vi "Test Day Total.vi"(8 "error in":errorcluster, 10 "Work Folder":path, 11 "Test Data Folder":path) -> (0 "error out":errorcluster, 2 "Report":string, 3 "Passed":bool)   [LabVIEW 2026]
doc: "Tests Day Total.vi and Day Total Entries.vi. Times are given as LOCAL date/time text and scanned here, so the daylight saving cases assume the US Central time zone of this computer (2026-11-01 has 25 hours, 2026-03-08 has 23).\n\nDay Total (entries built here): two finished entries add up; an entry crossing the next midnight counts only up to midnight; one started the previous evening counts only from midnight; a running entry counts up to Now and a later Now gives a larger total; overlapping entries are summed; 59.6 s rounds to 00:01:00 and 59 s stays 00:00:59; more than 24 h (overlaps) gives 25:00:00; on the 25-hour and the 23-hour day an entry from 00:00 to 23:59:59 and an entry spanning the whole day are clipped correctly; Now before the start counts 0; empty Entries gives 0 and 00:00:00.\n\nDay Total Entries (Test - Day Total Entries Cases.vi, on a copy of Test Data\\Samples with three entries added): an entry crossing local midnight is in the next day; the previous day is read from the previous month's file; a running entry from the previous day is included; the day's own entries come in start order; on the day after the 23-hour day 2026-03-08 (whose 24-hour read reaches into the next day) the entry is listed once; Day Total of each day's Total Entries; no error.\n\nInputs: Test Data Folder; Work Folder; error in. Outputs: Passed; Report; error out.\n\nGenerated by: Claude"
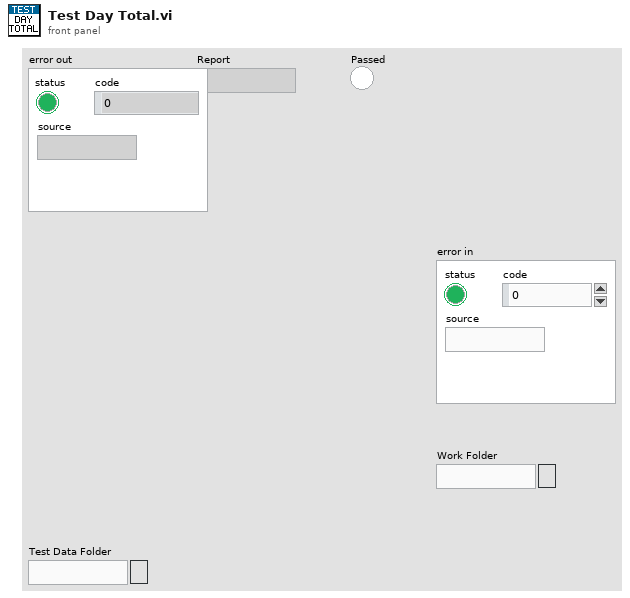
[diagram p1: front panel]
types:
  T1 = cluster{"ID":string, "Project ID":string, "Task ID":string, "Start Time":timestamp, "End Time":timestamp, "Description":string}
  T2 = cluster{"ID":string, "Project ID":string, "Task ID":string, "Start Time":timestamp, "End Time":timestamp, "Description":string}[]
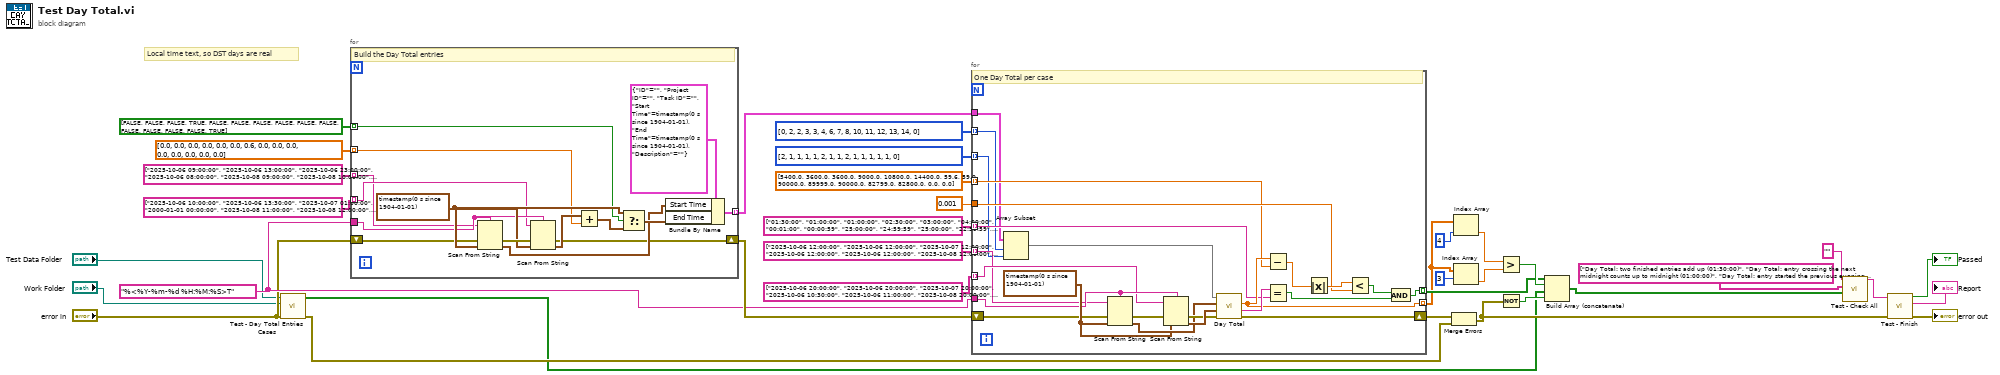
[diagram p0: block diagram]
diagram:
  w7 = "%<%Y-%m-%d %H:%M:%S>T" ("local time format")
  # "Local time text, so DST days are real"
  n1 = call "Test - Day Total Entries Cases.vi"("error in"="error in", "Work Folder"="Work Folder", "Test Data Folder"="Test Data Folder") -> ("error out"=w32:errorcluster, "Conditions"=w31:bool[])  [unwired: 7 in]
  n2 = for {
    tunnel: string[] ["2025-10-06 09:00:00", "2025-10-06 13:00:00", "2025-10-06 23:00:00", "2025-10-06 08:00:00", "2025-10-08 09:00:00", "2025-10-08 10:00:00", "2025-10-09 09:00:00", "2025-10-09 09:00:00", "2025-10-10 00:00:00", "2025-10-10 23:00:00", "2026-11-01 00:00:00", "2026-10-31 20:00:00", "2026-03-08 00:00:00", "2026-03-07 20:00:00", "2025-10-06 12:00:00"] ("entry starts") -> [w37] mode=indexing
    tunnel: string[] ["2025-10-06 10:00:00", "2025-10-06 13:30:00", "2025-10-07 01:00:00", "2000-01-01 00:00:00", "2025-10-08 11:00:00", "2025-10-08 12:00:00", "2025-10-09 09:00:59", "2025-10-09 09:00:59", "2025-10-11 00:00:00", "2025-10-11 00:00:00", "2026-11-01 23:59:59", "2026-11-02 04:00:00", "2026-03-08 23:59:59", "2026-03-09 04:00:00", "2000-01-01 00:00:00"] ("entry ends") -> [w38] mode=indexing
    tunnel: dbl[] [0.0, 0.0, 0.0, 0.0, 0.0, 0.0, 0.6, 0.0, 0.0, 0.0, 0.0, 0.0, 0.0, 0.0, 0.0] ("end extra seconds") -> [w39] mode=indexing
    tunnel: w7 -> [w40]
    tunnel: bool[] [FALSE, FALSE, FALSE, TRUE, FALSE, FALSE, FALSE, FALSE, FALSE, FALSE, FALSE, FALSE, FALSE, FALSE, TRUE] ("entry running") -> [w41] mode=indexing
    shift-right: [w43] -> w23
    shift-left: "error in" -> [w42]
    tunnel: [w51] -> w24 mode=indexing
    w45 = timestamp(0 s since 1904-01-01) ("default time")
    # "Build the Day Total entries"
    n3 = Scan From String(format string=w40, input string=w37, error in=w42, default 1=w45) -> (error out=w46:errorcluster, output 1=w47:timestamp)  [unwired: 1 in, 2 out]
    n4 = Scan From String(format string=w40, input string=w38, error in=w46, default 1=w45) -> (error out=w43:errorcluster, output 1=w48:timestamp)  [unwired: 1 in, 2 out]
    n5 = Add(x=w48, y=w39) -> (x+y=w49:timestamp)
    n6 = Select(t=w45, s=w41, f=w49) -> (s? t:f=w50:timestamp)
    n7 = Bundle By Name(cluster=T1 {"ID"="", "Project ID"="", "Task ID"="", "Start Time"=timestamp(0 s since 1904-01-01), "End Time"=timestamp(0 s since 1904-01-01), "Description"=""} ("entry"), "Start Time"=w47, "End Time"=w50) -> (w51:T1)
  }
  n8 = for {
    tunnel: i32[] [0, 2, 2, 3, 3, 4, 6, 7, 8, 10, 11, 12, 13, 14, 0] ("case first entry") -> [w52] mode=indexing
    tunnel: i32[] [2, 1, 1, 1, 1, 2, 1, 1, 2, 1, 1, 1, 1, 1, 0] ("case entry count") -> [w53] mode=indexing
    tunnel: string[] ["2025-10-06 12:00:00", "2025-10-06 12:00:00", "2025-10-07 12:00:00", "2025-10-06 12:00:00", "2025-10-06 12:00:00", "2025-10-08 12:00:00", "2025-10-09 12:00:00", "2025-10-09 12:00:00", "2025-10-10 12:00:00", "2026-11-01 12:00:00", "2026-11-01 12:00:00", "2026-03-08 12:00:00", "2026-03-08 12:00:00", "2025-10-06 12:00:00", "2025-10-06 12:00:00"] ("case days") -> [w54] mode=indexing
    tunnel: string[] ["2025-10-06 20:00:00", "2025-10-06 20:00:00", "2025-10-07 20:00:00", "2025-10-06 10:30:00", "2025-10-06 11:00:00", "2025-10-08 20:00:00", "2025-10-09 20:00:00", "2025-10-09 20:00:00", "2025-10-10 20:00:00", "2026-11-01 20:00:00", "2026-11-01 20:00:00", "2026-03-08 20:00:00", "2026-03-08 20:00:00", "2025-10-06 11:00:00", "2025-10-06 20:00:00"] ("case nows") -> [w55] mode=indexing
    tunnel: w7 -> [w57]
    tunnel: dbl[] [5400.0, 3600.0, 3600.0, 9000.0, 10800.0, 14400.0, 59.6, 59.0, 90000.0, 89999.0, 90000.0, 82799.0, 82800.0, 0.0, 0.0] ("expected seconds") -> [w58] mode=indexing
    tunnel: string[] ["01:30:00", "01:00:00", "01:00:00", "02:30:00", "03:00:00", "04:00:00", "00:01:00", "00:00:59", "25:00:00", "24:59:59", "25:00:00", "22:59:59", "23:00:00", "00:00:00", "00:00:00"] ("expected texts") -> [w59] mode=indexing
    tunnel: 0.001 ("tolerance s") -> [w60]
    shift-right: [w62] -> w25
    shift-left: w23 -> [w61]
    tunnel: w24 -> [w56]
    tunnel: [w69] -> w26 mode=indexing
    tunnel: [w75] -> w27 mode=indexing
    w63 = timestamp(0 s since 1904-01-01) ("default time")
    # "One Day Total per case"
    n9 = Array Subset(array=w56, index=w52, length=w53) -> (w68:T2)
    n10 = Scan From String(format string=w57, input string=w54, error in=w61, default 1=w63) -> (error out=w64:errorcluster, output 1=w65:timestamp)  [unwired: 1 in, 2 out]
    n11 = Scan From String(format string=w57, input string=w55, error in=w64, default 1=w63) -> (error out=w66:errorcluster, output 1=w67:timestamp)  [unwired: 1 in, 2 out]
    n12 = call "Day Total.vi"("error in"=w66, "Now"=w67, "Day"=w65, "Entries"=w68) -> ("error out"=w62:errorcluster, "Total Text"=w70:string, "Total Seconds"=w69:dbl)  [unwired: 5 in]
    n13 = Subtract(x=w69, y=w58) -> (x-y=w71:dbl)
    n14 = Equal?(x=w70, y=w59) -> (x = y?=w74:bool)
    n15 = Absolute Value(x=w71) -> (abs(x)=w72:dbl)
    n16 = Less?(x=w72, y=w60) -> (x < y?=w73:bool)
    n17 = And(x=w73, y=w74) -> (x .and. y?=w75:bool)
  }
  n18 = Merge Errors(w25, w32) -> (w33:errorcluster)
  n19 = Index Array(array=w26, index=4 ("later Now case")) -> (element=w29:dbl)
  n20 = Index Array(array=w26, index=3 ("earlier Now case")) -> (element=w28:dbl)
  n21 = Greater?(x=w29, y=w28) -> (0:w30:bool)
  n22 = Not(x=w33) -> (.not. x?=w34:bool)
  n23 = Build Array (concatenate)(w27, w30, w31, w34) -> (w35:bool[])
  n24 = call "Test - Check All.vi"("Conditions"=w35, "Check Names"=string[] ["Day Total: two finished entries add up (01:30:00)", "Day Total: entry crossing the next midnight counts up to midnight (01:00:00)", "Day Total: entry started the previous evening counts from midnight (01:00:00)", "Day Total: running entry counts up to Now (02:30:00)", "Day Total: running entry with a later Now (03:00:00)", "Day Total: overlapping entries are summed (04:00:00)", "Day Total: 59.6 s rounds to 00:01:00", "Day Total: 59 s gives 00:00:59", "Day Total: more than 24 h of overlaps gives 25:00:00", "Day Total: 25-hour day 2026-11-01 entry 00:00 to 23:59:59 gives 24:59:59", "Day Total: 25-hour day 2026-11-01 whole day gives 25:00:00", "Day Total: 23-hour day 2026-03-08 entry 00:00 to 23:59:59 gives 22:59:59", "Day Total: 23-hour day 2026-03-08 whole day gives 23:00:00", "Day Total: Now before the start counts 0", "Day Total: empty Entries gives 0 and 00:00:00", "Day Total: a later Now gives a larger total", "Day Total Entries: entry crossing local midnight is in the next day", "Day Total Entries: previous day read from the previous month file", "Day Total Entries: running entry from the previous day is included", "Day Total Entries: the day's own entries in start order", "Day Total Entries: listed once after the 23-hour day 2026-03-08", "Day Total Entries + Day Total: 2025-10-15 gives 01:30:00", "Day Total Entries + Day Total: 2025-11-01 gives 00:30:00", "Day Total Entries + Day Total: 2025-11-04 running from midnight gives 02:00:00", "Day Total Entries + Day Total: 2025-11-03 gives 04:38:59", "Day Total Entries + Day Total: 2026-03-09 gives 00:15:00", "Day Total and Day Total Entries: no error"] ("check names"), "Report in"="" ("empty report")) -> ("Report out"=w36:string)  [unwired: 7 in, 1 out]
  n25 = call "Test - Finish.vi"("error in (no error)"=w33, "Report"=w36) -> ("error out"=→"error out":errorcluster, "Report out"=→"Report":string, "Passed"=→"Passed":bool)  [unwired: 7 in]
